vi "usbpt104Open.vi"(1 "IP Address:port number":string="192.168.1.30:6250", 5 "Serial Number":string, 7 "Use Serial Number":bool, 8 "error in (no error)":errorcluster, 9 "Enumerate USB/Ethernet/ALL":u32(ring)=4294967295 items=["USB"=1, "Ethernet"=2, "ALL"=4294967295], 10 "Connection":bool=TRUE) -> (0 "error out":errorcluster, 2 "Unit Info":T1, 3 "handle out":i16=16384, 4 "PT-104 Units":string, 6 "serialLth":u32=13)   [LabVIEW 2010]
doc: "This VI manages listing and opens devices with device details."
uses:
  UsbPT104.dll
panel:
  # "USB"
  # "Ethernet"
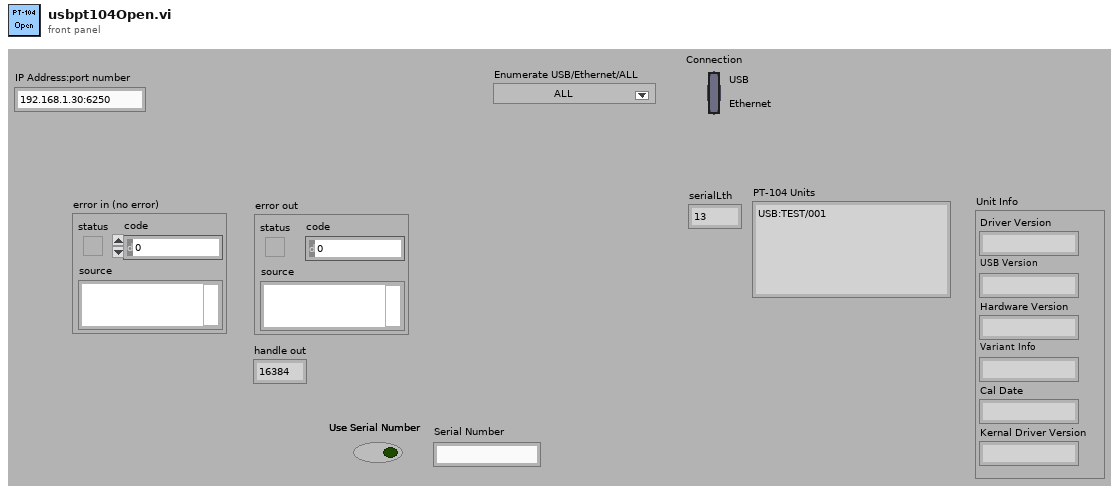
[diagram p1: front panel]
types:
  T1 = cluster{"Driver Version":string, "USB Version":string, "Hardware Version":string, "Variant Info":string, "Cal Date":string, "Kernal Driver Version":string, "NA":string, "NA 2":string, "NA":string, "NA 3":string, "NA 4":string, "NA 5":string, "NA 6":string, "NA 7":string, "NA 8":string}
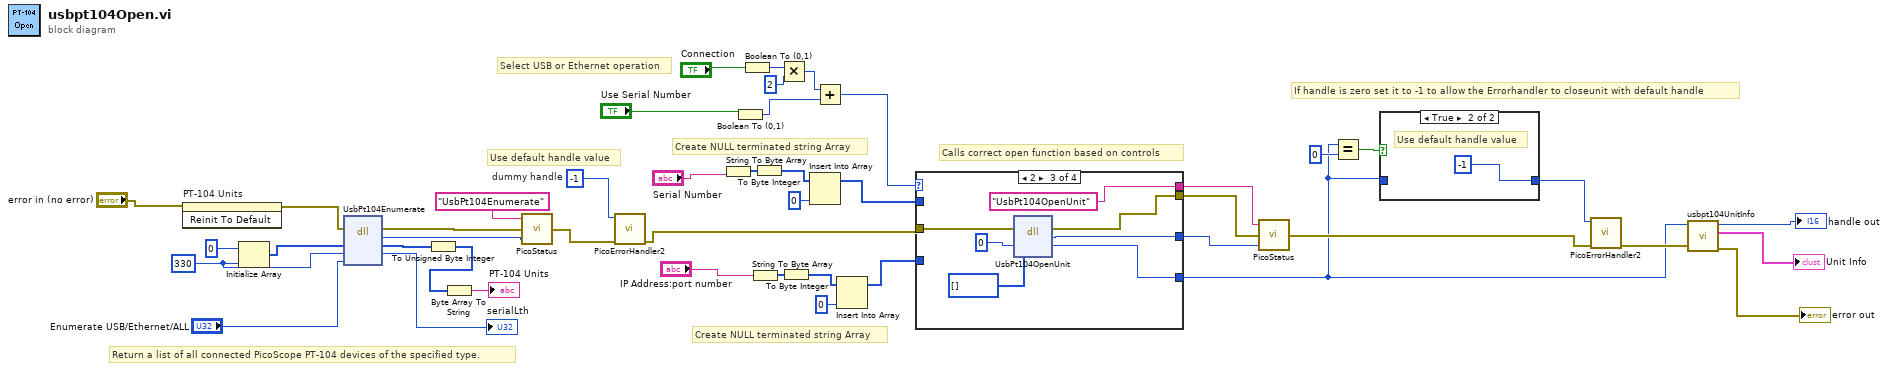
[diagram p0: block diagram]
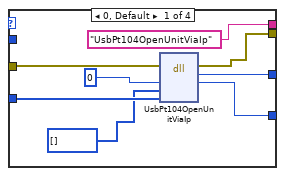
[diagram p3: hidden frame]
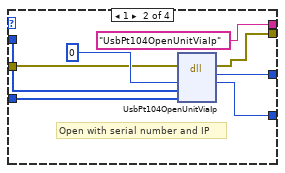
[diagram p4: hidden frame]
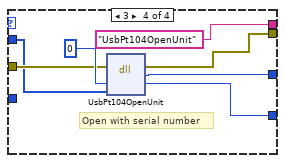
[diagram p5: hidden frame]
diagram:
  w5 = i16 -1  # dummy handle
  w27 = u32 330 ("dimension size")
  # "If handle is zero set it to -1 to allow the Errorhandler to closeunit with default handle"
  # "Calls correct open function based on controls"
  # "Use default handle value"
  # "Create NULL terminated string Array"
  # "Create NULL terminated string Array"
  # "Return a list of all connected PicoScope PT-104 devices of the specified type."
  # "Select USB or Ethernet operation"
  n1 = invoke on="PT-104 Units" class="Str" method="Reinit To Default"(error in="error in (no error)") -> (error out=w24:errorcluster)  [unwired: 2 in, 2 out]
  n2 = Initialize Array(i8 0 ("U8"), w27) -> (w29:i8[])
  n3 = dll-call lib="UsbPT104.dll" fn="UsbPt104Enumerate"(error in=w24, "details_str"=w29, "length"=w27, "type"="Enumerate USB/Ethernet/ALL") -> (error out=w34:errorcluster, "PICO_STATUS"=w33:u32, "details_str"=w25:i8[], "length"=→"serialLth":u32)  [unwired: 3 in, 1 out]
  n4 = To Unsigned Byte Integer(number=w25) -> (unsigned 8bit integer=w26:u8[])
  n5 = Byte Array To String(unsigned byte array=w26) -> (string=→"PT-104 Units":string)
  n6 = call "PicoStatus.vi"("PICO STATUS"=w33, "error in"=w34, "source"="UsbPt104Enumerate") -> ("error out"=w6:errorcluster)
  n7 = call "PicoErrorHandler2.vi"("error in (no error)"=w6, "handle In"=w5) -> ("error out"=w7:errorcluster)  [unwired: 9 in]
  n8 = String To Byte Array(string="Serial Number") -> (unsigned byte array=w13:u8[])
  n9 = Boolean To (0,1)(Boolean="Use Serial Number") -> (0, 1=w41:i16)
  n10 = Boolean To (0,1)(Boolean="Connection") -> (0, 1=w44:i16)
  n11 = String To Byte Array(string="IP Address:port number") -> (unsigned byte array=w18:u8[])
  n12 = To Byte Integer(number=w13) -> (8bit integer=w12:i8[])
  n13 = Multiply(x=w44, y=i16 2) -> (x*y=w42:i16)
  n14 = To Byte Integer(number=w18) -> (8bit integer=w17:i8[])
  n15 = Insert Into Array(array=w12, new element=i8 0 ("new element/subarray")) -> (w9:i8[])  [unwired: 1 in]
  n16 = Add(x=w42, y=w41) -> (x+y=w40:i16)
  n17 = Insert Into Array(array=w17, new element=i8 0 ("new element/subarray")) -> (w14:i8[])  [unwired: 1 in]
  n18 = case shown="2" w40 {
    tunnel: [w53 w60 w68 w75] -> w19
    tunnel: [w52 w59 w66 w73] -> w1
    tunnel: [w51 w58 w67 w74] -> w21
    tunnel: w7 -> [w50 w57 w64 w71]
    tunnel: w9 -> [_ w56 _ w70]
    tunnel: w14 -> [w49 w55 _ _]
    tunnel: ["UsbPt104OpenUnitViaIp" ("source") "UsbPt104OpenUnitViaIp" ("source") "UsbPt104OpenUnit" ("source") "UsbPt104OpenUnit" ("source")] -> w8
    frame 0, Default {
      n19 = dll-call lib="UsbPT104.dll" fn="UsbPt104OpenUnitViaIp"(error in=w50, "handle"=i16 0, "serial"=i8[] [], "IpAddress"=w49) -> (error out=w51:errorcluster, "PICO_STATUS"=w53:u32, "handle"=w52:i16)  [unwired: 4 in, 1 out]
    }
    frame 1 {
      # "Open with serial number and IP"
      n20 = dll-call lib="UsbPT104.dll" fn="UsbPt104OpenUnitViaIp"(error in=w57, "handle"=i16 0, "serial"=w56, "IpAddress"=w55) -> (error out=w58:errorcluster, "PICO_STATUS"=w60:u32, "handle"=w59:i16)  [unwired: 4 in, 1 out]
    }
    frame 2 {
      n21 = dll-call lib="UsbPT104.dll" fn="UsbPt104OpenUnit"(error in=w64, "handle"=i16 0, "serial"=i8[] []) -> (error out=w67:errorcluster, "PICO_STATUS"=w68:u32, "handle"=w66:i16)  [unwired: 3 in, 1 out]
    }
    frame 3 {
      # "Open with serial number"
      n22 = dll-call lib="UsbPT104.dll" fn="UsbPt104OpenUnit"(error in=w71, "handle"=i16 0, "serial"=w70) -> (error out=w74:errorcluster, "PICO_STATUS"=w75:u32, "handle"=w73:i16)  [unwired: 3 in, 1 out]
    }
  }
  n23 = call "PicoStatus.vi"("PICO STATUS"=w19, "error in"=w21, "source"=w8) -> ("error out"=w20:errorcluster)
  n24 = Equal?(x=w1, y=i16 0) -> (x = y?=w2:bool)
  n25 = case shown="True" w2 {
    tunnel: [w76 i16 -1 ("handle In")] -> w4
    tunnel: w1 -> [w76 _]
    frame False {
    }
    frame True {
      # "Use default handle value"
    }
  }
  n26 = call "PicoErrorHandler2.vi"("error in (no error)"=w20, "handle In"=w4) -> ("error out"=w22:errorcluster)  [unwired: 9 in]
  n27 = call "usbpt104UnitInfo.vi"("error in (no error)"=w22, "handle in"=w1) -> ("error out"=→"error out":errorcluster, "Unit Info"=→"Unit Info":T1, "handle out"=→"handle out":i16)  [unwired: 7 in]
